vi "Example - Hello Properties.vi"() -> ()   [LabVIEW 2019]
uses:
  src/KoRE-MQTT.lvlib
  src/KoRE-MQTT/Public/TypeDefs/MQTT Property - CONNECT.ctl
  src/KoRE-MQTT/Public/TypeDefs/MQTT Property - Will.ctl
  src/KoRE-MQTT/Public/TypeDefs/MQTT Property - PUBLISH.ctl
  src/KoRE-MQTT/Public/TypeDefs/MQTT Property Type.ctl
  src/KoRE-MQTT/Public/TypeDefs/MQTT Version.ctl
panel:
  out "error out":errorcluster
  out "Publish Properties Received (V5)":T1[](array[typedef]) {"Property" items=[" Payload Format Indicator          "=1, " Message Expiry Interval           "=2, " Content Type                      "=3, " Response Topic                    "=8, " Correlation Data                  "=9, " Subscription Identifier           "=11, " Topic Alias                       "=35, " User Property                     "=38]}
  in  "Version":T2=5 items=["3.11"=4, "5.0"=5]
  out "Sent?":bool
  in  "Port":u16=1883
  in  "Password":string
  in  "Username":string
  out "Received topic":string
  out "Received?":bool
  out "Send to topic":string
  out "Received message":string
  in  "Message":string="123.456"
  in  "Host":string(combo)="test.mosquitto.org"
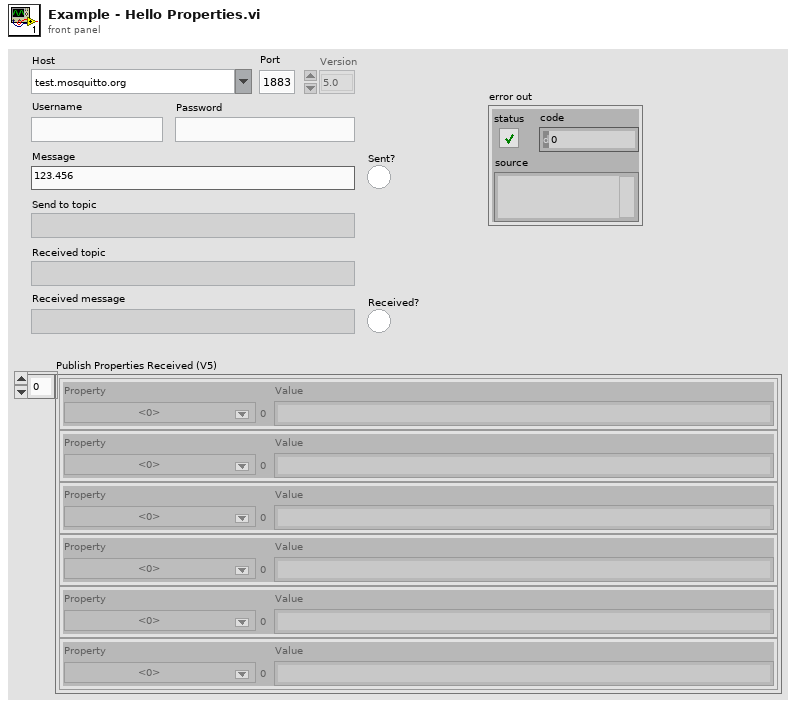
[diagram p1: front panel]
types:
  T1 = typedef "KoRE-MQTT.lvlib/MQTT Property - PUBLISH.ctl" = cluster{"Property":u8, "Value":string}
  T2 = typedef "KoRE-MQTT.lvlib/MQTT Version.ctl" = u16
  T3 = typedef "KoRE-MQTT.lvlib/MQTT Property Type.ctl" = u8
  T4 = typedef "KoRE-MQTT.lvlib/MQTT Property - Will.ctl" = cluster{"Property":u8, "Value":string}
  T5 = typedef "KoRE-MQTT.lvlib/MQTT Property - CONNECT.ctl" = cluster{"Property":u8, "Value":string}
  T6 = typedef "KoRE-MQTT.lvlib/MQTT Client Session.ctl" = refnum<vi>
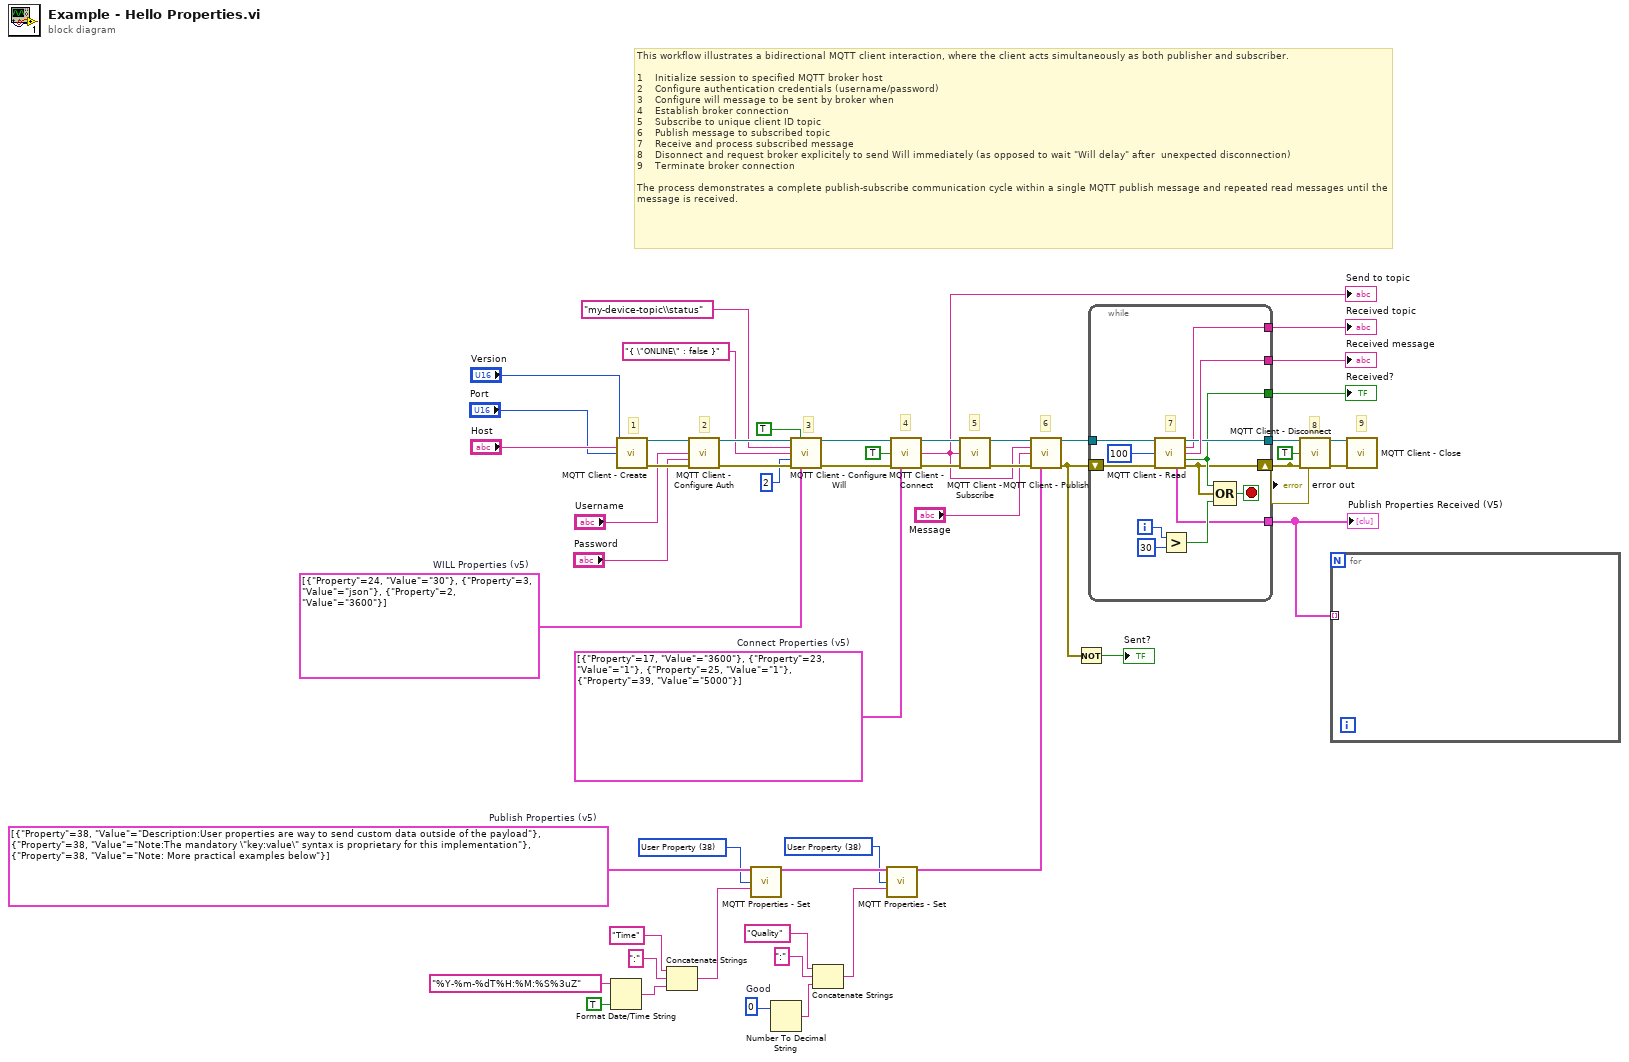
[diagram p0: block diagram]
diagram:
  w2 = 0  # Good
  w6 = T3 38 items=["Payload Format Indicator"=1, "Message Expiry Interval"=2, "Content Type"=3, "Response Topic"=8, "Correlation Data"=9, "Subscription Identifier"=11, "Session Expiry Interval"=17, "Assigned Client Identifier"=18, "Server Keep Alive"=19, "Authentication Method"=21, "Authentication Data"=22, "Request Problem Information"=23, "Will Delay Interval"=24, "Request Response Information"=25, "Response Information"=26, "Server Reference"=28, "Reason String"=31, "Receive Maximum"=33, "Topic Alias Maximum"=34, "Topic Alias"=35, "Maximum QoS"=36, "Retain Available"=37, "User Property"=38, "Maximum Packet Size"=39, "Wildcard Subscription Available"=40, "Subscription Identifier Available"=41, "Shared Subscription Available"=42] ("MQTT Property Type")
  w15 = T3 38 items=["Payload Format Indicator"=1, "Message Expiry Interval"=2, "Content Type"=3, "Response Topic"=8, "Correlation Data"=9, "Subscription Identifier"=11, "Session Expiry Interval"=17, "Assigned Client Identifier"=18, "Server Keep Alive"=19, "Authentication Method"=21, "Authentication Data"=22, "Request Problem Information"=23, "Will Delay Interval"=24, "Request Response Information"=25, "Response Information"=26, "Server Reference"=28, "Reason String"=31, "Receive Maximum"=33, "Topic Alias Maximum"=34, "Topic Alias"=35, "Maximum QoS"=36, "Retain Available"=37, "User Property"=38, "Maximum Packet Size"=39, "Wildcard Subscription Available"=40, "Subscription Identifier Available"=41, "Shared Subscription Available"=42] ("MQTT Property Type")
  w16 = T1[] [{"Property"=38, "Value"="Description:User properties are way to send custom data outside of the payload"}, {"Property"=38, "Value"="Note:The mandatory \"key:value\" syntax is proprietary for this implementation"}, {"Property"=38, "Value"="Note: More practical examples below"}]  # Publish Properties (v5)
  w22 = T4[] [{"Property"=24, "Value"="30"}, {"Property"=3, "Value"="json"}, {"Property"=2, "Value"="3600"}]  # WILL Properties (v5)
  w32 = T5[] [{"Property"=17, "Value"="3600"}, {"Property"=23, "Value"="1"}, {"Property"=25, "Value"="1"}, {"Property"=39, "Value"="5000"}]  # Connect Properties (v5)
  # "9"
  # "8"
  # "6"
  # "5"
  # "This workflow illustrates a bidirectional MQTT client interaction, where the client acts simultaneously as both publisher and subscriber.\n\n1    Initialize session to specified MQTT broker host\n2    Configure authentication credentials (username/password)\n3    Configure will message to be sent by broker when \n4    Establish broker connection\n5    Subscribe to unique client ID topic\n6    Publish message to subscribed topic\n7    Receive and process subscribed message\n8    Disonnect and request broker explicitely to send Will immediately (as opposed to wait \"Will delay\" after  unexpected disconnection)\n9    Terminate broker connection\n\nThe process demonstrates a complete publish-subscribe communication cycle within a single MQTT publish message and repeated read messages until the message is received."
  # "4"
  # "3"
  # "2"
  # "1"
  n1 = Format Date/Time String(time format string (%c)="%Y-%m-%dT%H:%M:%S%3uZ", UTC format=TRUE) -> (date/time string=w12:string)  [unwired: 1 in]
  n2 = call "MQTT Client - Create.vi"("Version (3.11)"="Version", "Host"="Host", "Port (1883)"="Port") -> ("MQTT Session"=w39:T6, "error out"=w40:errorcluster)  [unwired: 11 in]
  n3 = Concatenate Strings("Time" ("string"), ":" ("string"), w12) -> (w9:string)
  n4 = call "MQTT Client - Configure Auth.vi"("MQTT Session"=w39, "Username"="Username", "Password"="Password", "error in (no error)"=w40) -> ("MQTT Session out"=w31:T6, "error out"=w30:errorcluster)  [unwired: 10 in]
  n5 = call "MQTT Properties - Set.vi"("MQTT Properties"=w16, "MQTT Property Type"=w15, "Value"=w9) -> ("MQTT Properties out"=w8:cluster{"Property":u8, "Value":string}[])  [unwired: 12 in]
  n6 = Number To Decimal String(number=w2) -> (decimal integer string=w3:string)  [unwired: 1 in]
  n7 = call "MQTT Client - Configure Will.vi"("MQTT Session"=w31, "Will Retain (False)"=TRUE, "Will Topic"="my-device-topic\\status", "Will Payload"="{ \"ONLINE\" : false }", "Will QoS (0)"=u8 2, "error in"=w30, "WILL Properties (v5)"=w22) -> ("MQTT Session out"=w28:T6, "error out"=w29:errorcluster)  [unwired: 7 in]
  n8 = Concatenate Strings("Quality" ("string"), ":" ("string"), w3) -> (w1:string)
  n9 = call "MQTT Properties - Set.vi"("MQTT Properties"=w8, "MQTT Property Type"=w6, "Value"=w1) -> ("MQTT Properties out"=w7:cluster{"Property":u8, "Value":string}[])  [unwired: 12 in]
  n10 = call "MQTT Client - Connect.vi"("MQTT Session"=w28, "Clean Start"=TRUE, "error in (no error)"=w29, "Connect Properties (v5)"=w32) -> ("MQTT Session out"=w52:T6, "Assigned Client Identifier"=w42:string, "error out"=w51:errorcluster)  [unwired: 7 in, 2 out]
  "Send to topic" <- w42
  n11 = call "MQTT Client - Subscribe.vi"("MQTT Session"=w52, "Single Topic Filter"=w42, "error in (no error)"=w51) -> ("MQTT Session out"=w48:T6, "error out"=w49:errorcluster)  [unwired: 11 in]
  n12 = call "MQTT Client - Publish.vi"("MQTT Session"=w48, "Topic"=w42, "Message"="Message", "error in"=w49, "Publish Properties (v5)"=w7) -> ("MQTT Session out"=w47:T6, "error out"=w34:errorcluster)  [unwired: 9 in]
  n13 = Not(x=w34) -> (.not. x?=→"Sent?":bool)
  n14 = while {
    shift-right: [w55] -> w26
    shift-left: w34 -> [w59]
    tunnel: w47 -> [w64]
    tunnel: [w61] -> w46
    tunnel: [w60] -> w27
    tunnel: [w56] -> w45
    tunnel: [w58] -> w41
    tunnel: [w53] -> w17
    i -> [w63]
    stop <- w54 stop-if-true
    # "7"
    n15 = call "MQTT Client - Read.vi"("MQTT Session"=w64, "timeout (global)"=100, "error in (no error)"=w59) -> ("MQTT Session out"=w60:T6, "Topic"=w58:string, "Message"=w61:string, "New message?"=w56:bool, "Publish Properties Received (V5)"=w53:T1[], "error out"=w55:errorcluster)  [unwired: 6 in, 1 out]
    n16 = Greater?(x=w63, y=30) -> (0:w57:bool)
    n17 = Compound Arithmetic op=OR(w56, w55, w57) -> (w54:bool)
  }
  "Received message" <- w46
  "Received?" <- w45
  "Received topic" <- w41
  "Publish Properties Received (V5)" <- w17
  "error out" <- w26
  n18 = call "MQTT Client - Disconnect.vi"("MQTT Session"=w27, "With Will (v5)"=TRUE, "error in (no error)"=w26) -> ("MQTT Session out"=w24:T6, "error out"=w25:errorcluster)  [unwired: 11 in]
  n19 = for {
    tunnel: w17 -> [_] mode=indexing
  }
  n20 = call "MQTT Client - Close.vi"("MQTT session"=w24, "error in (no error)"=w25) -> ()  [unwired: 13 in, 1 out]
